vi "Read.vi"(6 "Append Index":i32, 8 "error in (no error)":errorcluster, 11 "Data Save in":refnum<class "LV-Data.lvclass">) -> (0 "error out":errorcluster, 1 "Notes":string, 2 "Data (Dictionary)":T1[](array[typedef]), 3 "Data Save out":refnum<class "LV-Data.lvclass">, 5 "Path out":path)   [LabVIEW 2019, in "LV-Data.lvclass"]
uses:
  LV-Data.lvclass
  Typedefs/Dictionary--cluster.ctl
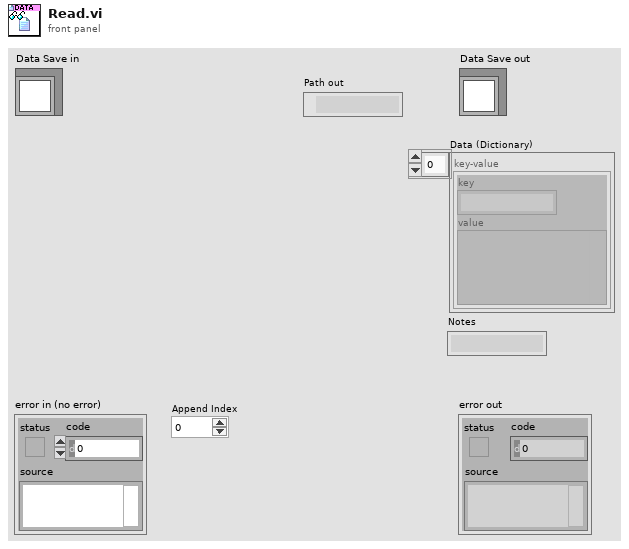
[diagram p1: front panel]
types:
  T1 = typedef "LV-Data.lvclass/Dictionary--cluster.ctl" = cluster{"key":string, "value":variant}
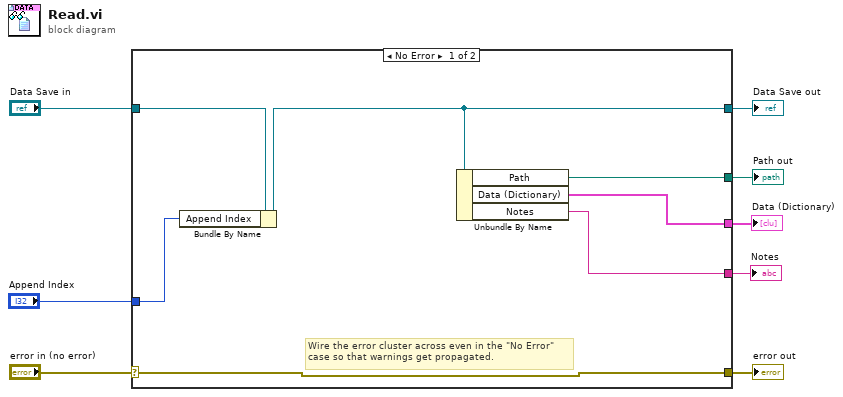
[diagram p0: block diagram]
diagram:
  n1 = case shown="No Error" "error in (no error)" {
    selector: "error in (no error)" -> [w10 w17]
    tunnel: [w10 w17] -> w7
    tunnel: [w13 w16] -> w5
    tunnel: "Data Save in" -> [w14 w16]
    tunnel: [w15 _] -> w4
    tunnel: [w9 _] -> w3
    tunnel: [w11 _] -> w2
    tunnel: "Append Index" -> [w12 _]
    frame No Error {
      # "Wire the error cluster across even in the \"No Error\"\ncase so that warnings get propagated."
      n2 = Bundle By Name(cluster=w14, "Append Index"=w12) -> (w13:refnum<class "LV-Data.lvclass">)
      n3 = Unbundle By Name(w13) -> ("Path"=w15:path, "Data (Dictionary)"=w9:T1[], "Notes"=w11:string)
    }
    frame Error {
    }
  }
  "error out" <- w7
  "Data Save out" <- w5
  "Path out" <- w4
  "Data (Dictionary)" <- w3
  "Notes" <- w2
